vi "Standard Normal.vi"() -> (3 "number":dbl)   [LabVIEW 2020, in "Full Featured MCP Server.lvlib"]
doc: "Returns a normally distributed random number with mean 0 and standard deviation 1 (Box-Muller method from two uniform random numbers)."
uses:
  Full Featured MCP Server.lvlib
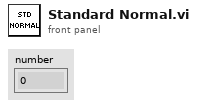
[diagram p1: front panel]
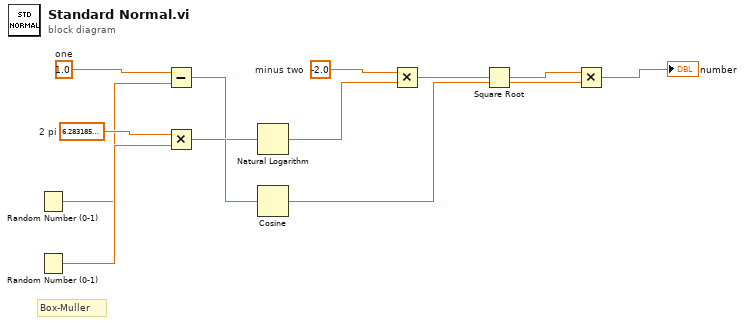
[diagram p0: block diagram]
diagram:
  w8 = 6.283185307179586  # 2 pi
  w4 = -2.0  # minus two
  w1 = 1.0  # one
  # "Box-Muller"
  n1 = Random Number (0-1)() -> (number: 0 to 1=w2:dbl)
  n2 = Random Number (0-1)() -> (number: 0 to 1=w9:dbl)
  n3 = Subtract(x=w1, y=w2) -> (x-y=w3:dbl)
  n4 = Multiply(x=w8, y=w9) -> (x*y=w10:dbl)
  n5 = Natural Logarithm(1:w3) -> (0:w5:dbl)
  n6 = Cosine(x=w10) -> (cos(x)=w11:dbl)
  n7 = Multiply(x=w4, y=w5) -> (x*y=w6:dbl)
  n8 = Square Root(x=w6) -> (sqrt(x)=w7:dbl)
  n9 = Multiply(x=w7, y=w11) -> (x*y=→"number":dbl)
